vi "FGV-GlobalEventQueues(lvlibp).vi"(6 "Create? (F)":bool, 8 "error in (no error)":errorcluster) -> (0 "error out":errorcluster, 2 "CreatedQueue":refnum<queue>, 3 "Queue":refnum<queue>[](array[refnum]))   [LabVIEW 2017, in "Communicable State Machine.lvlib"]
uses:
  Communicable State Machine.lvlib
  Typedef/_CSM_GlobalLog_MSG.ctl
  Typedef/_CSM_Response Source Message.ctl
  Typedef/_CSM_GlobalLog_MSG_TYPE.ctl
  FGV-GlobalEventQueues.vi
  _Shared/CSM Shared.lvlib
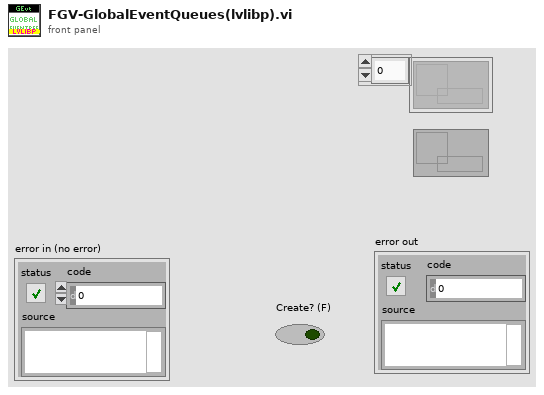
[diagram p1: front panel]
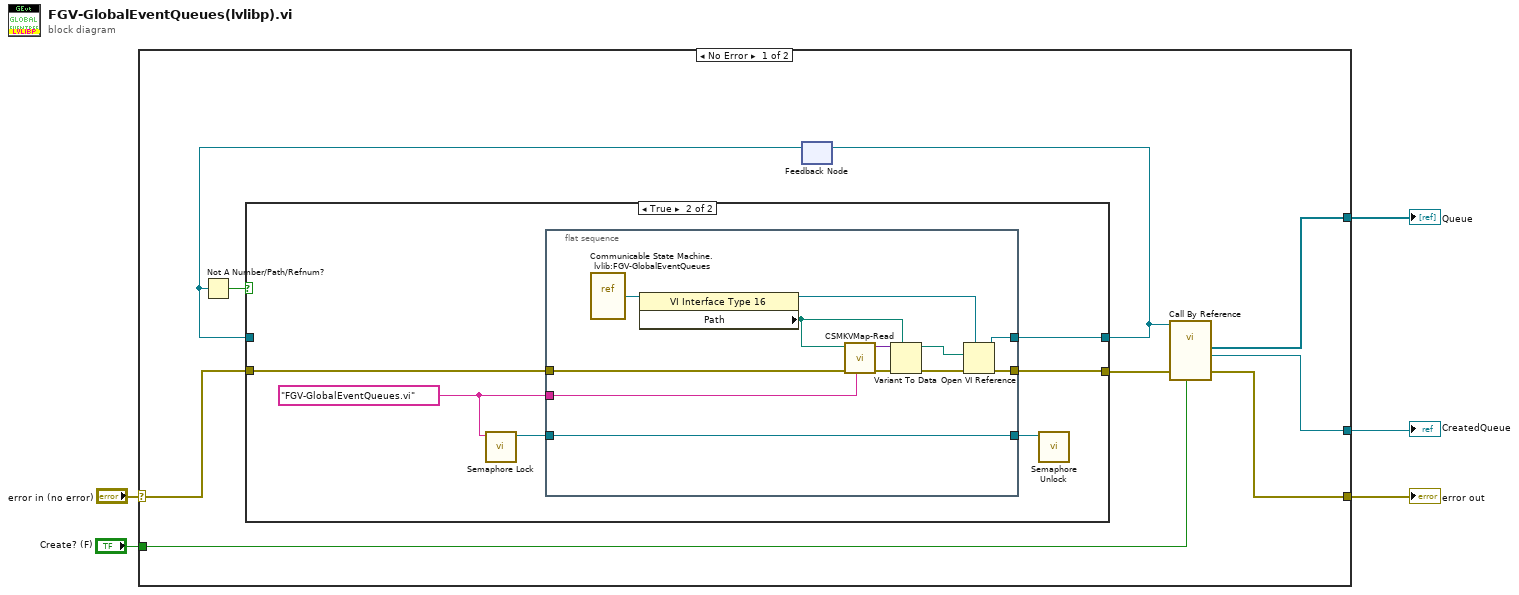
[diagram p0: block diagram]
diagram:
  n1 = case shown="No Error" "error in (no error)" {
    selector: "error in (no error)" -> [w10 w35]
    tunnel: [w8 _] -> w5
    tunnel: [w9 w35] -> w3
    tunnel: "Create? (F)" -> [w6 _]
    tunnel: [w7 _] -> w1
    frame No Error {
      n2 = feedback #1() -> (w13:refnum<vi>)  [unwired: 1 in]
      n3 = Not A Number/Path/Refnum?(number/path/refnum=w13) -> (NaN/Path/Refnum?=w14:bool)
      n4 = case shown="True" w14 {
        tunnel: [w15 w21] -> w12
        tunnel: [w16 w22] -> w11
        tunnel: w10 -> [w16 w20]
        tunnel: w13 -> [w15 _]
        frame False {
        }
        frame True {
          w19 = "FGV-GlobalEventQueues.vi" ("name")
          n5 = call "Semaphore Lock.vi"("name"=w19) -> ("semaphore"=w17:refnum<queue>)  [unwired: 10 in]
          n6 = flat-sequence {
            tunnel: [w30] -> w22
            tunnel: [w28] -> w21
            tunnel: w20 -> [w26]
            tunnel: w19 -> [w24]
            tunnel: [w23] -> w18
            tunnel: w17 -> [w23]
            frame #0 {
              n7 = vi-ref "Communicable State Machine.lvlib:FGV-GlobalEventQueues.vi"() -> (w25:refnum<vi>)
              n8 = property class="VI Interface Type 16"(reference=w25) -> (reference out=w27:refnum<vi>, "Path"=w29:path)  [unwired: 1 in, 1 out]
              n9 = call "CSMKVMap-Read.vi"("name"=w24, "Error in"=w26, "default value (empty variant)"=w29) -> ("Error out"=w34:errorcluster, "value"=w33:variant)  [unwired: 5 in]
              n10 = Variant To Data(error in=w34, type=w29, Variant=w33) -> (data=w32:path, error out=w31:errorcluster)
              n11 = Open VI Reference(type specifier VI Refnum (for type only)=w27, vi path=w32, error in (no error)=w31) -> (vi reference=w28:refnum<vi>, error out=w30:errorcluster)  [unwired: 3 in]
            }
          }
          n12 = call "Semaphore Unlock.vi"("semaphore"=w18) -> ()  [unwired: 11 in]
        }
      }
      n13 = feedback-in #1(w12) -> ()
      n14 = call-by-ref "?"(reference=w12, "Create? (F)"=w6, "error in (no error)"=w11) -> ("error out"=w9:errorcluster, "CreatedQueue"=w7:refnum<queue>, "Queue"=w8:refnum<queue>[])  [unwired: 8 in, 2 out]
    }
    frame Error {
    }
  }
  "Queue" <- w5
  "error out" <- w3
  "CreatedQueue" <- w1
